vi "RemoteVI Complex Fixture Value Text.vi"(0 "value":variant, 11 "error in":errorcluster) -> (4 "text":string, 15 "error out":errorcluster)   [LabVIEW 2020]
doc: "Event-log helper of RemoteVI Complex Fixture.vi. The text of a value of any type for a value line of the log: the contents of every Val element of LabVIEW's XML of the value (Flatten To XML), joined with |. A numeric gives its number, a string or path its text, a boolean 0 or 1, an enum or tab control its index, a cluster its elements in order (Name|Gain|Enabled), an array or table its elements row by row. error in is passed through unchanged."
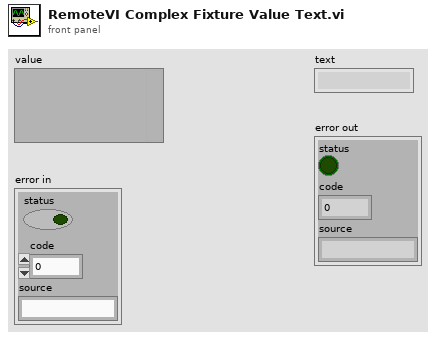
[diagram p1: front panel]
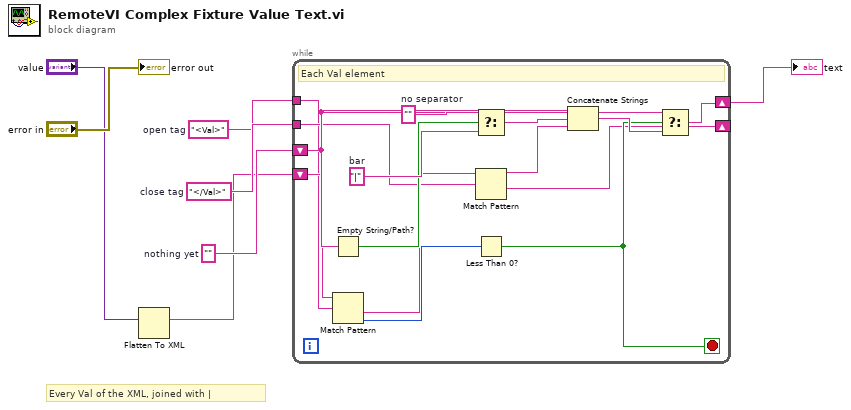
[diagram p0: block diagram]
diagram:
  w6 = ""  # nothing yet
  w5 = "</Val>"  # close tag
  w4 = "<Val>"  # open tag
  # "Every Val of the XML, joined with |"
  n1 = Flatten To XML(6:"value") -> (2:w3:string)
  n2 = while {
    tunnel: w4 -> [w8]
    tunnel: w5 -> [w9]
    shift-right: [w13] -> w7
    shift-left: w6 -> [w12]
    shift-right: [w11] -> _
    shift-left: w3 -> [w10]
    stop <- w18 stop-if-true
    w20 = "|"  # bar
    w17 = ""  # no separator
    # "Each Val element"
    n3 = Empty String/Path?(string/path=w12) -> (empty?=w19:bool)
    n4 = Match Pattern(string=w10, regular expression=w8) -> (after substring=w14:string, offset past match=w15:i32)  [unwired: 1 in, 2 out]
    n5 = Select(t=w17, s=w19, f=w20) -> (s? t:f=w21:string)
    n6 = Match Pattern(string=w14, regular expression=w9) -> (before substring=w16:string, after substring=w11:string)  [unwired: 1 in, 2 out]
    n7 = Less Than 0?(x=w15) -> (x < 0?=w18:bool)
    n8 = Concatenate Strings(w12, w21, w16) -> (w22:string)
    n9 = Select(t=w12, s=w18, f=w22) -> (s? t:f=w13:string)
  }
  "text" <- w7
  "error out" <- "error in"
